vi "test_brokenVITest.vi"(8 "error in (no error)":errorcluster, 11 "TestCase in":refnum<class "lvCICD_TestCase.lvclass">) -> (0 "error out":errorcluster, 3 "TestCase out":refnum<class "lvCICD_TestCase.lvclass">)   [LabVIEW 2014, in "lvCICD_TestCase.lvclass"]
uses:
  lvCICD_TestCase.lvclass
  <vilib>/addons/_JKI Toolkits/VI Tester/TestCase.llb/TestCase.lvclass
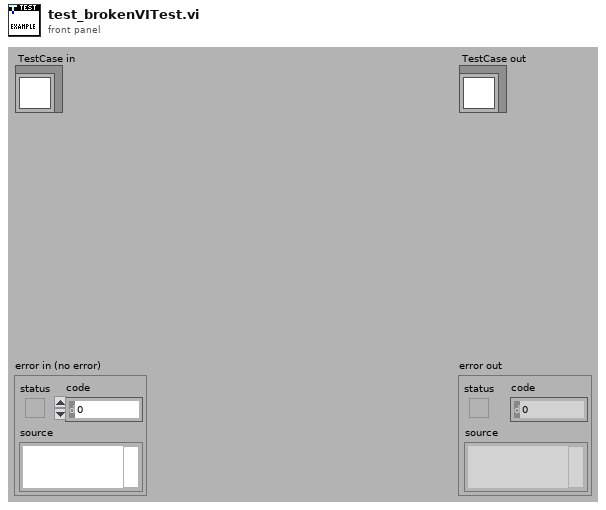
[diagram p1: front panel]
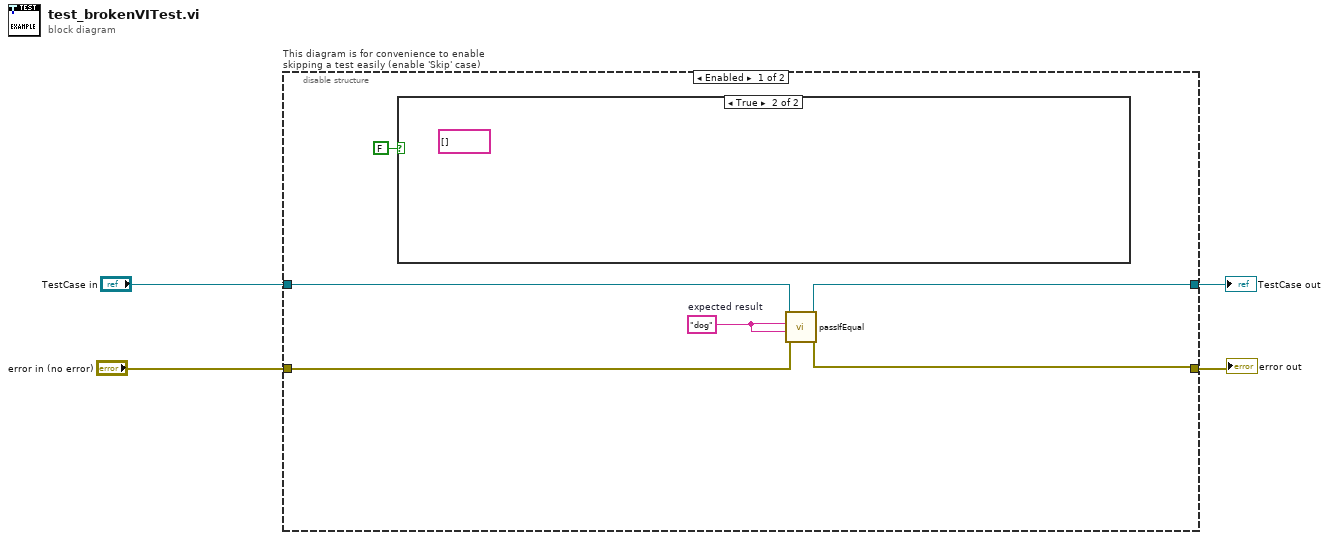
[diagram p0: block diagram]
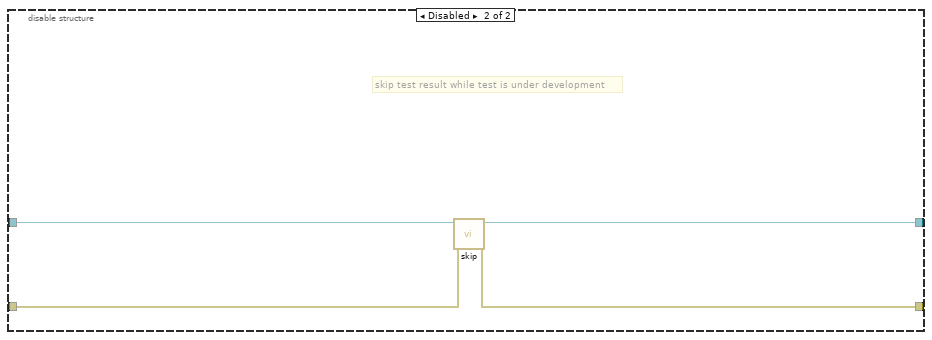
[diagram p3: hidden frame]
diagram:
  n1 = disable-structure "This diagram is for convenience to enable skipping a test easily (enable 'Skip' case)" shown="Enabled" {
    disable-tunnel: "TestCase in" -> [w10 w14]
    disable-tunnel: [w9 w12] -> w1
    disable-tunnel: [w8 w13] -> w3
    disable-tunnel: "error in (no error)" -> [w7 w11]
    frame Enabled {
      w6 = "dog"  # expected result
      n2 = case shown="True" FALSE {
        frame False {
        }
        frame True {
          (unwired) string[] [] ("CommandLine")
        }
      }
      n3 = call-dynamic "passIfEqual.vi"("error in (no error)"=w7, "y"=w6, "x"=w6, "TestCase in"=w10) -> ("error out"=w8:errorcluster, "TestCase out"=w9:refnum<class "lvCICD_TestCase.lvclass">)  [unwired: 6 in]
    }
    frame Disabled {
      # "skip test result while test is under development"
      n4 = call <vilib>:"skip.vi"("error in (no error)"=w11, "TestCase in"=w14) -> ("error out"=w13:errorcluster, "TestCase out"=w12:refnum<class "lvCICD_TestCase.lvclass">)  [unwired: 8 in]
    }
  }
  "error out" <- w3
  "TestCase out" <- w1
